vi "ERW-IoT MATLAB Batch.vi"() -> ()   [LabVIEW 2026]
panel:
  out "MATLAB output":string
  in  "MATLAB demo command":string="/Users/tejasshandilya/Documents/Codex/2026-10-12/x/outputs/ERW-IoT/run_matlab_demo.sh"
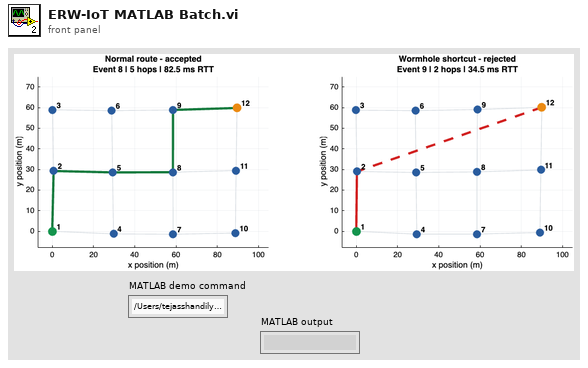
[diagram p1: front panel]
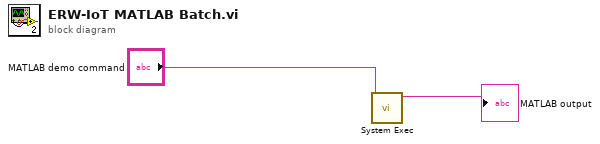
[diagram p0: block diagram]
diagram:
  n1 = call <vilib>:"System Exec.vi"("standard input"="MATLAB demo command", "command line"="MATLAB demo command") -> ("standard output"=→"MATLAB output":string)  [unwired: 6 in, 3 out]
